vi "TCP Send Image.vi"(0 "Connection ID":refnum<k5>, 7 "Image Stack (U16)":u16[][][](array[numeric]), 11 "Error In":errorcluster) -> (4 "Connection ID Out":refnum<k5>, 8 "Success?":bool, 15 "Error Out":errorcluster)   [LabVIEW 2016]
panel:
  out "Image Size":i32[](array[numeric])
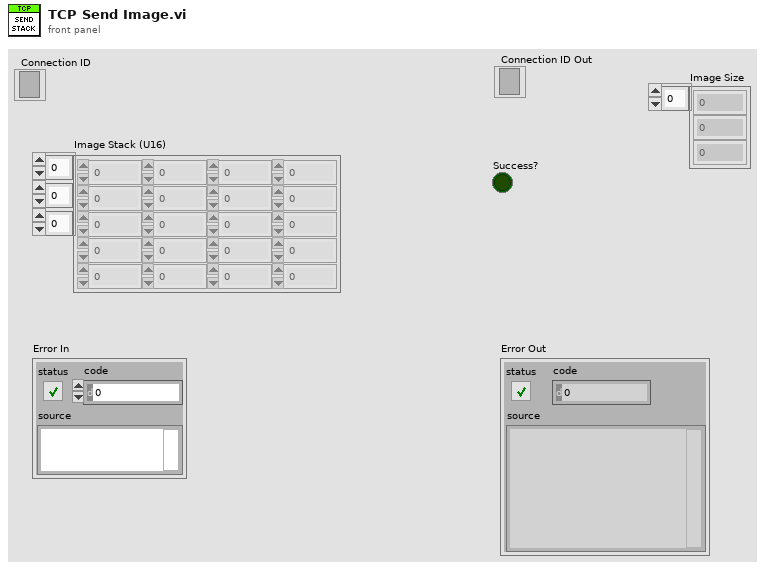
[diagram p1: front panel]
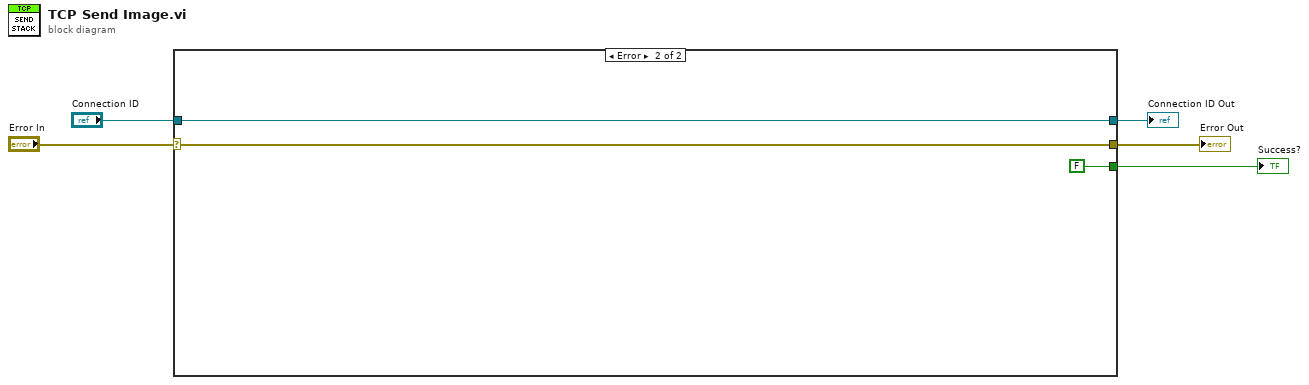
[diagram p0: block diagram]
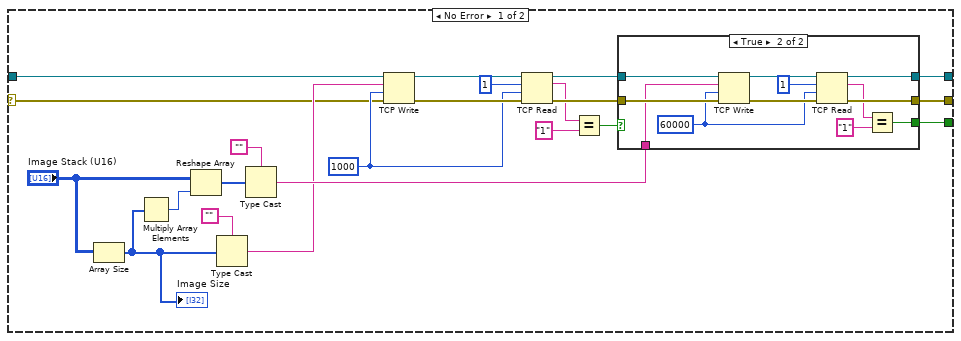
[diagram p2: hidden frame]
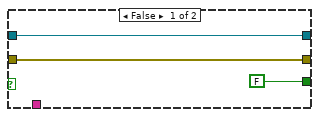
[diagram p3: hidden frame]
diagram:
  n1 = case shown="Error" "Error In" {
    selector: "Error In" -> [w6 w44]
    tunnel: "Connection ID" -> [w25 w45]
    tunnel: [w22 w45] -> w4
    tunnel: [w17 w44] -> w3
    tunnel: [w10 FALSE] -> w2
    frame No Error {
      w11 = 1000 ("timeout ms (25000)")
      n2 = Array Size(array="Image Stack (U16)") -> (size(s)=w9:i32[])
      "Image Size" <- w9
      n3 = Multiply Array Elements(1:w9) -> (0:w20:i32)
      n4 = Reshape Array("Image Stack (U16)", w20) -> (w27:u16[])
      n5 = Type Cast(type="", x=w9) -> (*(type *) &x=w8:string)
      n6 = Type Cast(type="", x=w27) -> (*(type *) &x=w12:string)
      n7 = TCP Write(connection ID=w25, data in=w8, error in (no error)=w6, 9:w11) -> (connection ID out=w24:refnum<k5>, error out=w19:errorcluster)  [unwired: 1 out]
      n8 = TCP Read(connection ID=w24, bytes to read=1, error in (no error)=w19, 9:w11) -> (connection ID out=w23:refnum<k5>, data out=w14:string, error out=w18:errorcluster)  [unwired: 1 in]
      n9 = Equal?(x=w14, y="1") -> (x = y?=w13:bool)
      n10 = case shown="True" w13 {
        tunnel: w23 -> [w30 w42]
        tunnel: [w30 w40] -> w22
        tunnel: w18 -> [w29 w39]
        tunnel: [w29 w37] -> w17
        tunnel: w12 -> [_ w36]
        tunnel: [FALSE w32] -> w10
        frame False {
        }
        frame True {
          w31 = 60000 ("timeout ms (25000)")
          n11 = TCP Write(connection ID=w42, data in=w36, error in (no error)=w39, 9:w31) -> (connection ID out=w41:refnum<k5>, error out=w38:errorcluster)  [unwired: 1 out]
          n12 = TCP Read(connection ID=w41, bytes to read=1, error in (no error)=w38, 9:w31) -> (connection ID out=w40:refnum<k5>, data out=w33:string, error out=w37:errorcluster)  [unwired: 1 in]
          n13 = Equal?(x=w33, y="1") -> (x = y?=w32:bool)
        }
      }
    }
    frame Error {
    }
  }
  "Connection ID Out" <- w4
  "Error Out" <- w3
  "Success?" <- w2
